vi "lvgit commit.vi"(8 "error in":errorcluster, 11 "path":path) -> (0 "error out":errorcluster)   [LabVIEW 2017]
panel:
  out "Staged Files":string[](array[string])
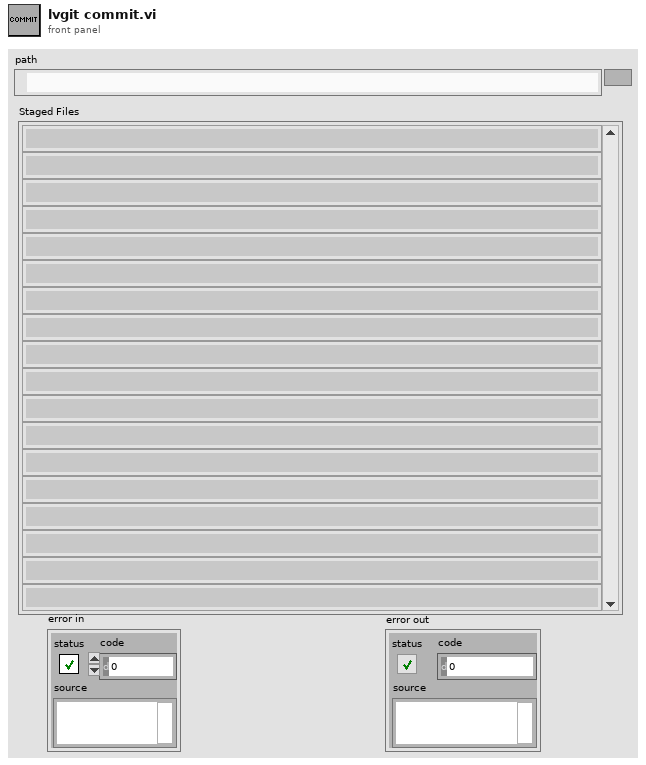
[diagram p1: front panel]
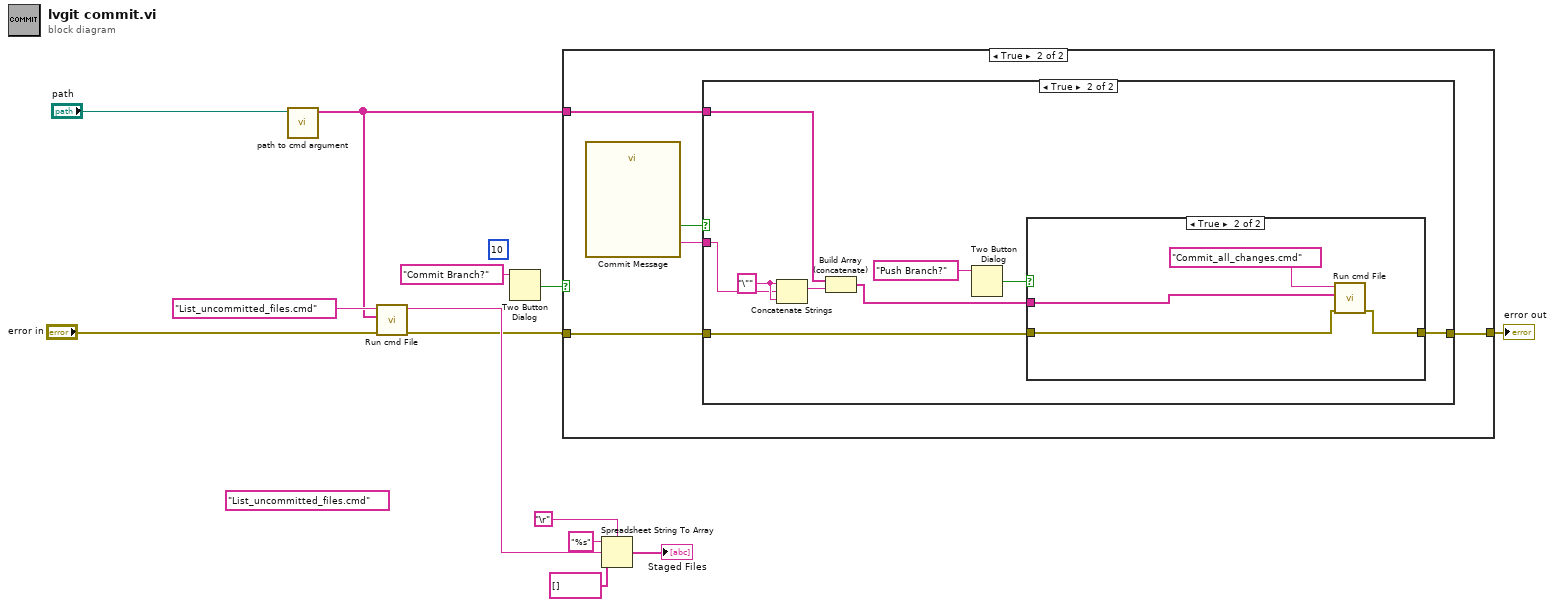
[diagram p0: block diagram]
diagram:
  (unwired) "List_uncommitted_files.cmd" ("name or relative path")
  (unwired) 10 ("F Timeout(-1 s)")
  n1 = call "path to cmd argument.vi"("path"="path") -> ("Array"=w1:string[])  [unwired: 10 in]
  n2 = call "Run cmd File.vi"("Error in"="error in", "args"=w1, "name or relative path"="List_uncommitted_files.cmd") -> ("Error out"=w4:errorcluster, "standard output"=w9:string)  [unwired: 6 in, 1 out]
  n3 = Two Button Dialog(message="Commit Branch?") -> (T button?=w12:bool)  [unwired: 2 in]
  n4 = case shown="True" w12 {
    tunnel: [w14 w17] -> w11
    tunnel: w4 -> [w14 w16]
    tunnel: w1 -> [_ w15]
    frame False {
    }
    frame True {
      n5 = call "Commit Message"() -> ("Message"=w19:string, "OK"=w18:bool)  [unwired: 17 in, 1 out]
      n6 = case shown="True" w18 {
        tunnel: [w20 w28] -> w17
        tunnel: w16 -> [w20 w29]
        tunnel: w19 -> [_ w23]
        tunnel: w15 -> [_ w22]
        frame False {
        }
        frame True {
          w25 = "\"" ("string")
          n7 = Concatenate Strings(w25, w23, w25) -> (w24:string)
          n8 = Build Array (concatenate)(w22, w24) -> (w21:string[])
          n9 = Two Button Dialog(message="Push Branch?") -> (T button?=w26:bool)  [unwired: 2 in]
          n10 = case shown="True" w26 {
            tunnel: w29 -> [w30 w34]
            tunnel: [w30 w33] -> w28
            tunnel: w21 -> [_ w31]
            frame False {
            }
            frame True {
              n11 = call "Run cmd File.vi"("Error in"=w34, "args"=w31, "name or relative path"="Commit_all_changes.cmd") -> ("Error out"=w33:errorcluster)  [unwired: 6 in, 2 out]
            }
          }
        }
      }
    }
  }
  "error out" <- w11
  n12 = Spreadsheet String To Array(delimiter (Tab)="\r", format string="%s", spreadsheet string=w9, array type (2D Dbl)=string[] [] ("Array of Strings")) -> (array=→"Staged Files":string[])
